vi "Caracterizacion_wn_zeta.vi"() -> ()   [LabVIEW 2021]
uses:
  <vilib>/DAQmx/read.llb/DAQmx Read (Counter DBL 1Chan 1Samp).vi
  <vilib>/DAQmx/create/channels.llb/DAQmx Create Channel (CI-Position-Angular Encoder).vi
  <vilib>/DAQmx/miscellaneous.llb/DAQmx Fill In Error Info.vi
  <vilib>/Utility/file.llb/Write Delimited Spreadsheet (DBL).vi
  <resource>/objmgr/daqmx.rc
panel:
  in  "V motor [V]":dbl
  out "ang":dbl
  out "dbg_g":dbl
  out "dbg_H":dbl
  out "dirO":dbl
  out "extO":dbl
  out "textO":dbl
  out "lastO":dbl
  in  "Archivo de logs":path=path "C:/Users/labfisica/Documents/Codigo_Proyecto_Pendulo-main/Logs/resultados_motor2.txt.txt"
  out "Recorridos":i32[](array[numeric])
  out "Tiempos de pico":dbl[](array[numeric])
  out "delta":dbl
  out "Td [s]":dbl
  out "wn [rad/s]":dbl
  out "zeta":dbl
  in  "counter":tag="Dev1/ctr0"
  out "Válido":bool
  out "Posición [°]":dbl(graph)
  in  "stop":bool
  in  "Tiempo max [s]":dbl=60.0
  in  "minRun":dbl=20.0
  in  "H":dbl=3.0
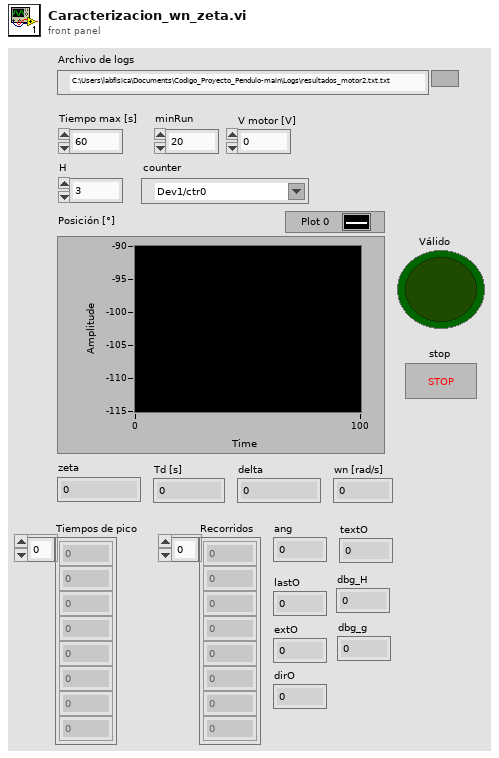
[diagram p1: front panel]
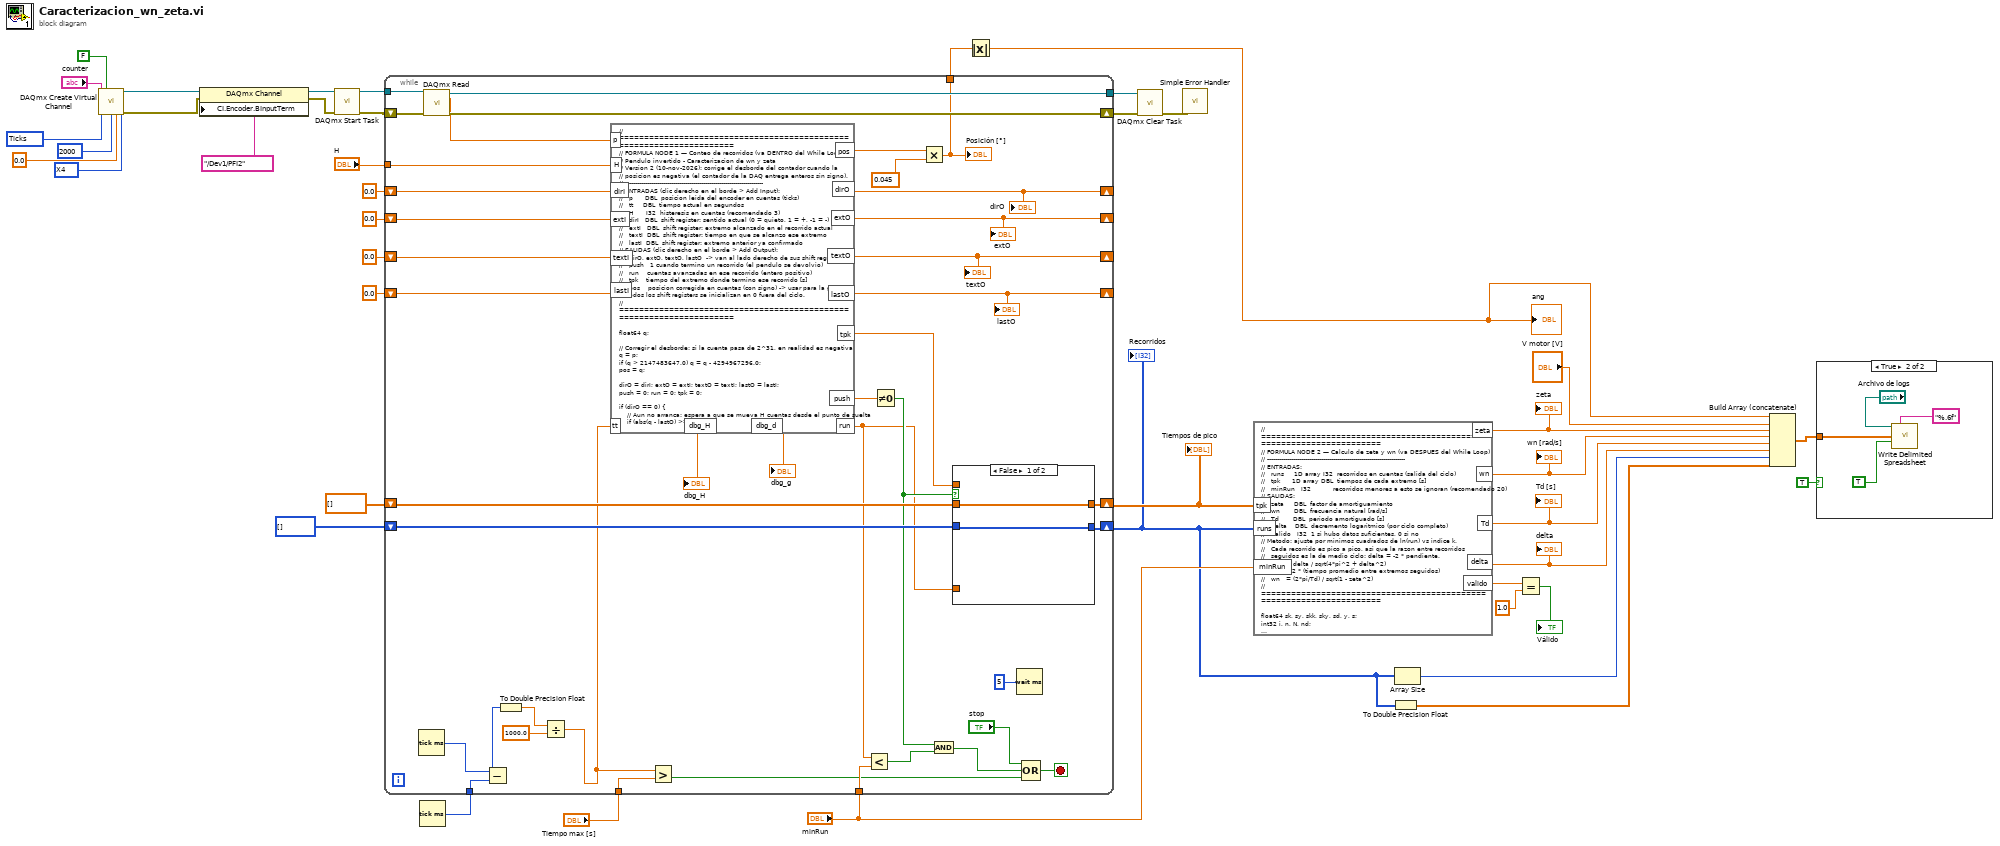
[diagram p0: block diagram]
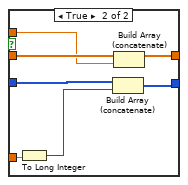
[diagram p3: hidden frame]
diagram:
  w39 = 10304 items=["Degrees"=10146, "Radians"=10273, "Ticks"=10304, "From Custom Scale"=10065] ("units")
  w41 = 10092 items=["X1"=10090, "X2"=10091, "X4"=10092, "Two Pulse Counting"=10313] ("decoding type")
  n1 = call-poly <vilib>:"DAQmx Create Virtual Channel.vi"("z index enable"=FALSE, "counter"="counter", "decoding type"=w41, "units"=w39, "pulses per revolution"=u32 2000, "initial angle"=0.0) -> ("task out"=w12:refnum<k21>, "error out"=w11:errorcluster)  [unwired: 8 in]
  n2 = property class="DAQmx Channel"(reference=w12, error in=w11, "CI.Encoder.BInputTerm"=tag "/Dev1/PFI2") -> (reference out=w10:refnum<k21>, error out=w9:errorcluster)
  n3 = call <vilib>:"DAQmx Start Task.vi"("task/channels in"=w10, "error in"=w9) -> ("task out"=w37:refnum<k21>, "error out"=w36:errorcluster)  [unwired: 12 in]
  n4 = Tick Count (ms)() -> (millisecond timer value=w35:u32)
  n5 = while {
    shift-right: [w72] -> _
    shift-left: 0.0 ("extO") -> [w73]
    shift-right: [w81] -> w27
    shift-left: w36 -> [w82]
    shift-right: [w71] -> _
    shift-left: 0.0 ("textO") -> [w70]
    shift-right: [w66] -> w4
    shift-left: i32[] [] -> [w64]
    shift-right: [w68] -> _
    shift-left: 0.0 ("lastO") -> [w69]
    shift-right: [w53] -> w20
    shift-left: dbl[] [] -> [w65]
    tunnel: w37 -> [w83]
    shift-right: [w74] -> _
    shift-left: 0.0 ("dirO") -> [w75]
    tunnel: w35 -> [w79]
    tunnel: "H" -> [w76]
    tunnel: "Tiempo max [s]" -> [w59]
    tunnel: "minRun" -> [w58]
    tunnel: [w55] -> w26
    tunnel: [w43] -> w5
    stop <- w56 stop-if-true
    n6 = Tick Count (ms)() -> (millisecond timer value=w80:u32)
    n7 = call-poly <vilib>:"DAQmx Read.vi"("task/channels in"=w83, "error in"=w82) -> ("task out"=w55:refnum<k21>, "data"=w62:dbl, "error out"=w81:errorcluster)  [unwired: 11 in]
    n8 = Subtract(x=w80, y=w79) -> (x-y=w78:u32)
    n9 = To Double Precision Float(number=w78) -> (double precision float=w48:dbl)
    n10 = Divide(x=w48, y=1000.0) -> (x/y=w54:dbl)
    n11 = formula code="// =====================================================================\n// FORMULA NODE 1 — Conteo de recorridos (va DENTRO del While Loop)\n// Pendulo invertido - Caracterizacion de wn y zeta\n// Version 2 (10-nov-2026): corrige el desborde del contador cuando la\n// posicion es negativa (el contador de la DAQ entrega enteros sin signo).\n// ---------------------------------------------------------------------\n// ENTRADAS (clic derecho en el borde > Add Input):\n//   p      DBL  posicion leida del encoder en cuentas (ticks)\n//   tt     DBL  tiempo actual en segundos\n//   H      I32  histeresis en cuentas (recomendado 3)\n//   dirI   DBL  shift register: sentido actual (0 = quieto, 1 = +, -1 = -)\n//   extI   DBL  shift register: extremo alcanzado en el recorrido actual\n//   textI  DBL  shift register: tiempo en que se alcanzo ese extremo\n//   lastI  DBL  shift register: extremo anterior ya confirmado\n// SALIDAS (clic derecho en el borde > Add Output):\n//   dirO, extO, textO, lastO  -> van al lado derecho de sus shift registers\n//   push   1 cuando termino un recorrido (el pendulo se devolvio)\n//   run    cuentas avanzadas en ese recorrido (entero positivo)\n//   tpk    tiempo del extremo donde termino ese recorrido [s]\n//   pos    posicion corregida en cuentas (con signo) -> usar para la grafica\n// Todos los shift registers se inicializan en 0 fuera del ciclo.\n// =====================================================================\n\nfloat64 q;\n\n// Corregir el desborde: si la cuenta pasa de 2^31, en realidad es negativa\nq = p;\nif (q > 2147483647.0) q = q - 4294967296.0;\npos = q;\n\ndirO = dirI; extO = extI; textO = textI; lastO = lastI;\npush = 0; run = 0; tpk = 0;\n\nif (dirO == 0) {\n    // Aun no arranca: espera a que se mueva H cuentas desde el punto de suelta\n    if (abs(q - lastO) >= H) {\n        if (q > lastO) dirO = 1; else dirO = -1;\n        extO = q; textO = tt;\n    }\n} else if (dirO == 1) {\n    // Avanzando en sentido +\n    if (q > extO) {\n        extO = q; textO = tt;\n    } else if (extO - q >= H) {\n        // Se devolvio: se cierra el recorrido\n        push = 1; run = extO - lastO; tpk = textO;\n        lastO = extO; dirO = -1; extO = q; textO = tt;\n    }\n} else {\n    // Avanzando en sentido -\n    if (q < extO) {\n        extO = q; textO = tt;\n    } else if (q - extO >= H) {\n        push = 1; run = lastO - extO; tpk = textO;\n        lastO = extO; dirO = 1; extO = q; textO = tt;\n    }\n}\ndbg_d = abs(q - lastI);\ndbg_H = H;"("p"=w62, "tt"=w54, "H"=w76, "dirI"=w75, "extI"=w73, "textI"=w70, "lastI"=w69) -> ("dirO"=w74:dbl, "extO"=w72:dbl, "textO"=w71:dbl, "lastO"=w68:dbl, "push"=w67:dbl, "run"=w47:dbl, "tpk"=w63:dbl, "pos"=w46:dbl, "dbg_d"=→"dbg_g":dbl, "dbg_H"=→"dbg_H":dbl)
    "lastO" <- w68
    "textO" <- w71
    "extO" <- w72
    "dirO" <- w74
    n12 = Greater?(x=w54, y=w59) -> (0:w52:bool)
    n13 = Less?(x=w47, y=w58) -> (x < y?=w50:bool)
    n14 = Not Equal To 0?(x=w67) -> (x != 0?=w57:bool)
    n15 = Multiply(x=w46, y=0.045) -> (x*y=w43:dbl)
    "Posición [°]" <- w43
    n16 = And(x=w57, y=w50) -> (x .and. y?=w51:bool)
    n17 = case shown="False" w57 {
      tunnel: w47 -> [_ w92]
      tunnel: w64 -> [w85 w91]
      tunnel: [w85 w89] -> w66
      tunnel: w65 -> [w84 w88]
      tunnel: w63 -> [_ w86]
      tunnel: [w84 w87] -> w53
      frame False {
      }
      frame True {
        n18 = To Long Integer(number=w92) -> (32bit integer=w90:i32)
        n19 = Build Array (concatenate)(w91, w90) -> (w89:i32[])
        n20 = Build Array (concatenate)(w88, w86) -> (w87:dbl[])
      }
    }
    n21 = Wait (ms)(milliseconds to wait=u32 5) -> ()  [unwired: 1 out]
    n22 = Compound Arithmetic op=OR("stop", w51, w52) -> (w56:bool)
  }
  "Tiempos de pico" <- w20
  "Recorridos" <- w4
  n23 = Absolute Value(x=w5) -> (abs(x)=w6:dbl)
  "ang" <- w6
  n24 = call <vilib>:"DAQmx Clear Task.vi"("task in"=w26, "error in"=w27) -> ("error out"=w25:errorcluster)  [unwired: 13 in]
  n25 = call <vilib>:"Simple Error Handler.vi"("error in (no error)"=w25) -> ()  [unwired: 4 in, 5 out]
  n26 = formula code="// =====================================================================\n// FORMULA NODE 2 — Calculo de zeta y wn (va DESPUES del While Loop)\n// ---------------------------------------------------------------------\n// ENTRADAS:\n//   runs     1D array I32  recorridos en cuentas (salida del ciclo)\n//   tpk      1D array DBL  tiempos de cada extremo [s]\n//   minRun   I32           recorridos menores a esto se ignoran (recomendado 20)\n// SALIDAS:\n//   zeta     DBL  factor de amortiguamiento\n//   wn       DBL  frecuencia natural [rad/s]\n//   Td       DBL  periodo amortiguado [s]\n//   delta    DBL  decremento logaritmico (por ciclo completo)\n//   valido   I32  1 si hubo datos suficientes, 0 si no\n// Metodo: ajuste por minimos cuadrados de ln(run) vs indice k.\n//   Cada recorrido es pico a pico, asi que la razon entre recorridos\n//   seguidos es la de medio ciclo: delta = -2 * pendiente.\n//   zeta = delta / sqrt(4*pi^2 + delta^2)\n//   Td   = 2 * (tiempo promedio entre extremos seguidos)\n//   wn   = (2*pi/Td) / sqrt(1 - zeta^2)\n// =====================================================================\n\nfloat64 sk, sy, skk, sky, sd, y, s;\nint32 i, n, N, nd;\n\nsk = 0; sy = 0; skk = 0; sky = 0; sd = 0;\nN = 0; nd = 0;\nn = sizeOfDim(runs, 0);\n\nfor (i = 0; i < n; i++) {\n    if (runs[i] >= minRun) {\n        y = ln(runs[i]);\n        sk = sk + i;  sy = sy + y;  skk = skk + i*i;  sky = sky + i*y;\n        N = N + 1;\n        if (i > 0) {\n            if (runs[i-1] >= minRun) {\n                sd = sd + (tpk[i] - tpk[i-1]);\n                nd = nd + 1;\n            }\n        }\n    }\n}\n\nif (N >= 3 && nd >= 1) {\n    s     = (N*sky - sk*sy) / (N*skk - sk*sk);\n    delta = -2*s;\n    zeta  = delta / sqrt(4*pi*pi + delta*delta);\n    Td    = 2*sd/nd;\n    wn    = (2*pi/Td) / sqrt(1 - zeta*zeta);\n    valido = 1;\n} else {\n    delta = 0; zeta = 0; Td = 0; wn = 0;\n    valido = 0;\n}"("runs"=w4, "tpk"=w20, "minRun"="minRun") -> ("zeta"=w16:dbl, "wn"=w18:dbl, "Td"=w15:dbl, "delta"=w14:dbl, "valido"=w23:dbl)
  "zeta" <- w16
  "wn [rad/s]" <- w18
  "Td [s]" <- w15
  "delta" <- w14
  n27 = To Double Precision Float(number=w4) -> (double precision float=w3:dbl[])
  n28 = Array Size(array=w4) -> (size(s)=w17:i32)
  n29 = Equal?(x=w23, y=1.0) -> (x = y?=→"Válido":bool)
  n30 = Build Array (concatenate)(w6, "V motor [V]", w16, w18, w15, w14, w17, w3) -> (w13:dbl[])
  n31 = case shown="True" TRUE {
    tunnel: w13 -> [_ w95]
    frame False {
    }
    frame True {
      n32 = call-poly <vilib>:"Write Delimited Spreadsheet.vi"("file path (dialog if empty)"="Archivo de logs", "format (%.3f)"="%.6f", "1D data"=w95, "append to file? (new file:F)"=TRUE) -> ()  [unwired: 10 in, 2 out]
    }
  }
